vi "delete tag.vi"(7 "owner ID":string, 8 "error in":errorcluster, 10 "tag name":string, 11 "engine configuration in":refnum<class "engine configuration.lvclass">) -> (0 "error out":errorcluster, 3 "engine configuration out":refnum<class "engine configuration.lvclass">)   [LabVIEW 2014, in "engine configuration.lvclass"]
doc: "This function deletes the tag from the engine configuration specified by 'tag name'. In deleting a tag, any mappings associated with that tag are also deleted.\n\nIf the tag was created by a specific owned, that owner must input its owner ID to this function. Only the owner of a tag is allowed to delete it."
uses:
  engine configuration.lvclass
  <vilib>/NI/Tag Bus/tag/tag descriptor.lvclass
  <vilib>/NI/Tag Bus/tag/tag descriptor.lvclass/tag descriptor.ctl
  engine configuration.lvclass/engine configuration.ctl
  <vilib>/NI/Tag Bus/tag/write tag name.vi
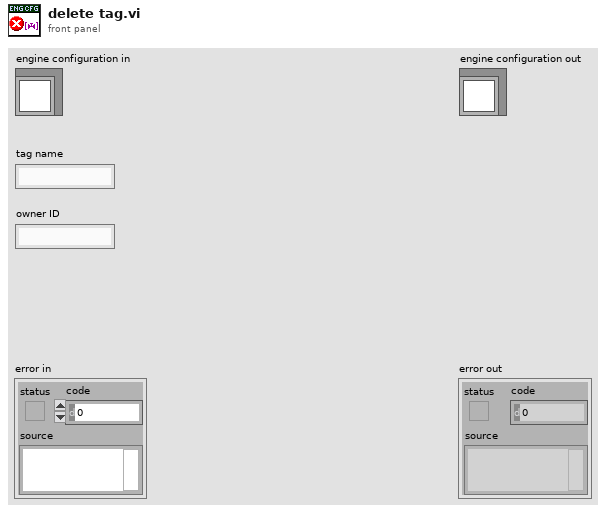
[diagram p1: front panel]
types:
  T1 = typedef "engine configuration.lvclass/module channel pairings.ctl" = cluster{"modules":string[], "channels":string[]}
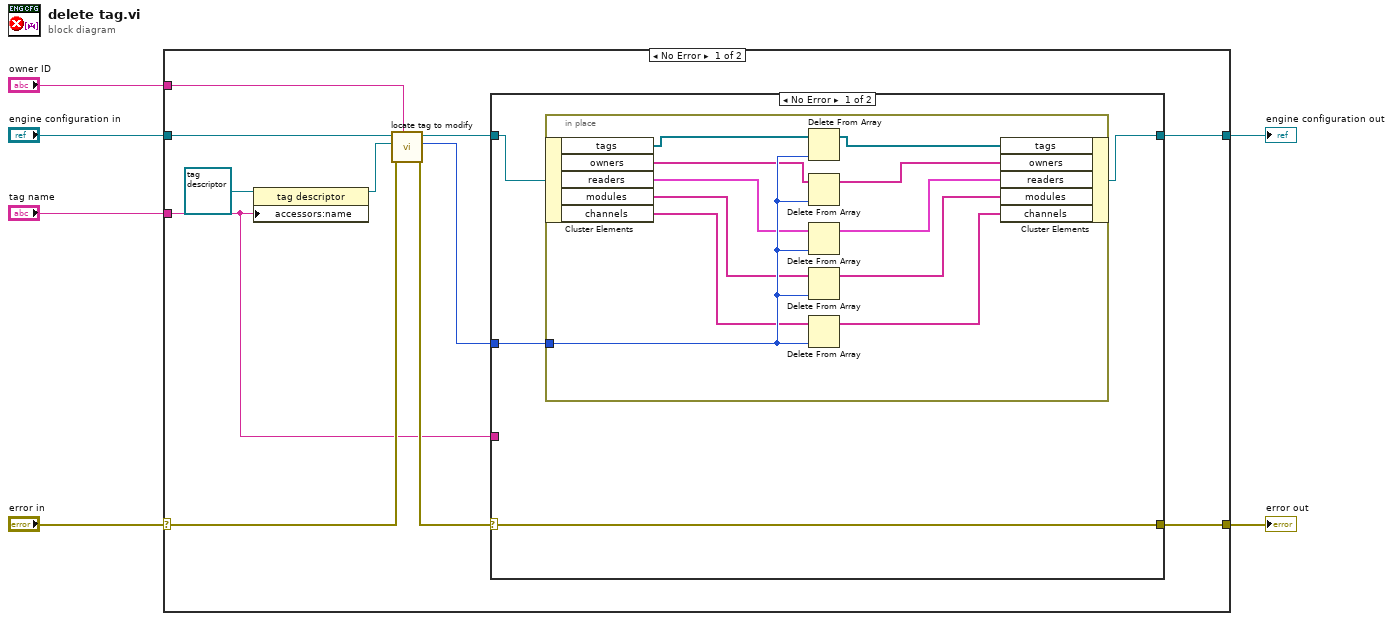
[diagram p0: block diagram]
diagram:
  n1 = case shown="No Error" "error in" {
    selector: "error in" -> [w11 w36]
    tunnel: [w16 w36] -> w2
    tunnel: [w17 w35] -> w3
    tunnel: "engine configuration in" -> [w15 w35]
    tunnel: "tag name" -> [w7 _]
    tunnel: "owner ID" -> [w14 _]
    frame No Error {
      n2 = property class="tag descriptor"(reference=refnum<class "tag descriptor.lvclass"> refnum ("tag descriptor"), "accessors:name"=w7) -> (reference out=w12:refnum<class "tag descriptor.lvclass">)  [unwired: 1 in, 1 out]
      n3 = call "locate tag to modify.vi"("owner ID"=w14, "error in"=w11, "tag descriptor"=w12, "engine configuration in"=w15) -> ("error out"=w9:errorcluster, "index"=w8:i32, "engine configuration out"=w10:refnum<class "engine configuration.lvclass">)  [unwired: 5 in]
      n4 = case shown="No Error" w9 {
        selector: w9 -> [w21 w33]
        tunnel: w10 -> [w20 w34]
        tunnel: [w18 w34] -> w17
        tunnel: [w21 w33] -> w16
        tunnel: w8 -> [w19 _]
        tunnel: w7 -> [_ _]
        frame No Error {
          n5 = in-place {
            in-place-border: w19 -> [w32]
            n6 = in-place-cluster #1(w20) -> ("tags"=w31:refnum<class "tag descriptor.lvclass">[], "owners"=w28:string[], "readers"=w27:T1[], "modules"=w22:string[], "channels"=w23:string[])
            n7 = Delete From Array(array=w31, index=w32) -> (array with subset deleted=w30:refnum<class "tag descriptor.lvclass">[])  [unwired: 1 in, 1 out]
            n8 = Delete From Array(array=w28, index=w32) -> (array with subset deleted=w29:string[])  [unwired: 1 in, 1 out]
            n9 = Delete From Array(array=w27, index=w32) -> (array with subset deleted=w26:T1[])  [unwired: 1 in, 1 out]
            n10 = Delete From Array(array=w22, index=w32) -> (array with subset deleted=w25:string[])  [unwired: 1 in, 1 out]
            n11 = Delete From Array(array=w23, index=w32) -> (array with subset deleted=w24:string[])  [unwired: 1 in, 1 out]
            n12 = in-place-cluster #1("tags"=w30, "owners"=w29, "readers"=w26, "modules"=w25, "channels"=w24) -> (w18:refnum<class "engine configuration.lvclass">)
          }
        }
        frame Error {
        }
      }
    }
    frame Error {
    }
  }
  "error out" <- w2
  "engine configuration out" <- w3
